vi "Copy Builds To NIVS Dir.vi"(5 "Files Generated by Build":path[](array[path]), 6 "Top Level/Always Included VIs":path[](array[path]), 7 "Destination Path":path, 8 "error in (no error)":errorcluster, 9 "Target Name":string, 10 "Build Specification Name":string, 11 "Project Path":path) -> (0 "error out":errorcluster)   [LabVIEW 2024]
uses:
  <vilib>/Utility/sysdir.llb/System Directory Type.ctl
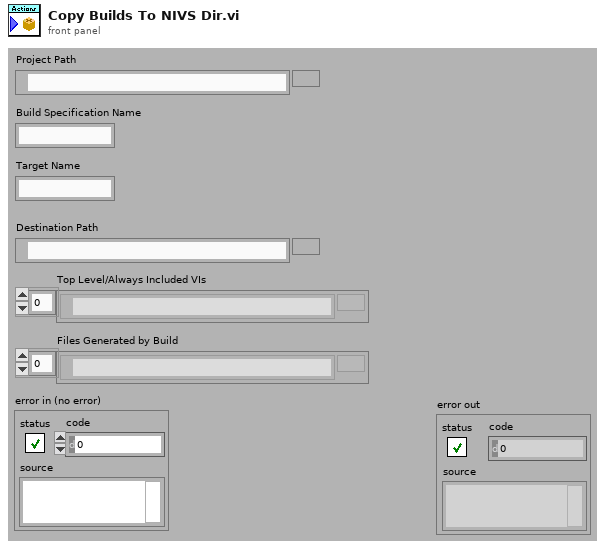
[diagram p1: front panel]
types:
  T1 = typedef "System Directory Type.ctl" = i32
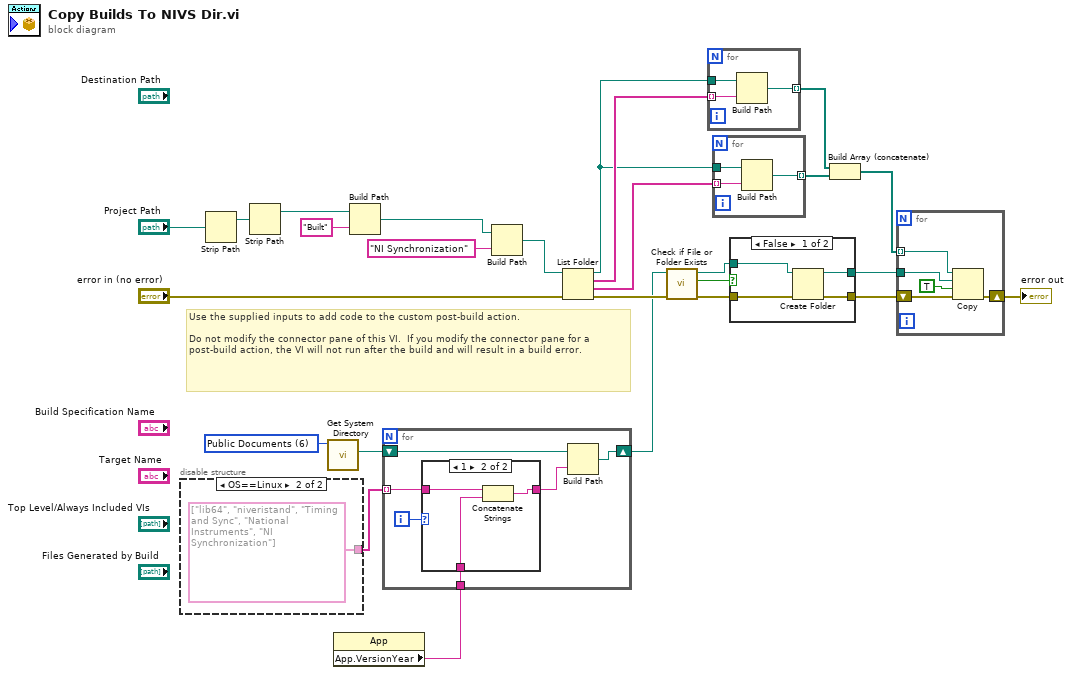
[diagram p0: block diagram]
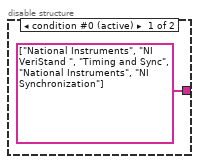
[diagram p2: hidden frame]
diagram:
  w7 = T1 6 items=["User Home"=0, "User Desktop"=1, "User Documents"=2, "User Application Data"=3, "User Preferences"=4, "User Temporary"=5, "Public Documents"=6, "Public Application Data"=7, "Public Preferences"=8, "Public Cache"=13, "System Core Libraries"=9, "System Installed Libraries"=10, "Application Files"=11, "Boot Volume Root"=12] ("system directory type")
  # "Use the supplied inputs to add code to the custom post-build action.\n\nDo not modify the connector pane of this VI.  If you modify the connector pane for a post-build action, the VI will not run after the build and will result in a build error."
  n1 = disable-structure shown="OS==Linux" {
    disable-tunnel: [string[] ["National Instruments", "NI VeriStand ", "Timing and Sync", "National Instruments", "NI Synchronization"] string[] ["lib64", "niveristand", "Timing and Sync", "National Instruments", "NI Synchronization"]] -> w5
    frame condition #0 (active) {
    }
    frame condition #1 {
    }
  }
  n2 = Strip Path(path="Project Path") -> (stripped path=w11:path)  [unwired: 1 out]
  n3 = Strip Path(path=w11) -> (stripped path=w22:path)  [unwired: 1 out]
  n4 = call <vilib>:"Get System Directory.vi"("system directory type"=w7) -> ("system directory"=w6:path)  [unwired: 10 in]
  n5 = property class="App"() -> ("App.VersionYear"=w3:string)  [unwired: 2 in, 2 out]
  n6 = Build Path(base path=w22, name or relative path="Built") -> (appended path=w2:path)
  n7 = for {
    shift-right: [w33] -> w4
    shift-left: w6 -> [w34]
    tunnel: w5 -> [w30] mode=indexing
    tunnel: w3 -> [w29]
    i -> [w32]
    n8 = case shown="1" w32 {
      tunnel: [w35 w37] -> w31
      tunnel: w30 -> [w35 w38]
      tunnel: w29 -> [_ w36]
      frame Default {
      }
      frame 1 {
        n9 = Concatenate Strings(w38, w36) -> (w37:string)
      }
    }
    n10 = Build Path(base path=w34, name or relative path=w31) -> (appended path=w33:path)
  }
  n11 = Build Path(base path=w2, name or relative path="NI Synchronization") -> (appended path=w10:path)
  n12 = List Folder(path=w10, error in="error in (no error)") -> (path out=w13:path, filenames=w26:string[], folder names=w14:string[], error out=w8:errorcluster)  [unwired: 2 in]
  n13 = call <vilib>:"Check if File or Folder Exists.vi"("error in (no error)"=w8, "path"=w4) -> ("error out"=w17:errorcluster, "file or folder exists?"=w19:bool, "dup path"=w18:path)  [unwired: 7 in]
  n14 = for {
    tunnel: w26 -> [w40] mode=indexing
    tunnel: w13 -> [w41]
    tunnel: [w39] -> w25 mode=indexing
    n15 = Build Path(base path=w41, name or relative path=w40) -> (appended path=w39:path)
  }
  n16 = for {
    tunnel: w14 -> [w43] mode=indexing
    tunnel: w13 -> [w44]
    tunnel: [w42] -> w12 mode=indexing
    n17 = Build Path(base path=w44, name or relative path=w43) -> (appended path=w42:path)
  }
  n18 = case shown="False" w19 {
    tunnel: w18 -> [w48 w50]
    tunnel: w17 -> [w47 w49]
    tunnel: [w46 w50] -> w16
    tunnel: [w45 w49] -> w15
    frame False {
      n19 = Create Folder(path (use dialog)=w48, error in=w47) -> (created path=w46:path, error out=w45:errorcluster)  [unwired: 1 in, 1 out]
    }
    frame True {
    }
  }
  n20 = Build Array (concatenate)(w25, w12) -> (w24:path[])
  n21 = for {
    tunnel: w24 -> [w52] mode=indexing
    shift-right: [w53] -> w1
    shift-left: w15 -> [w54]
    tunnel: w16 -> [w51]
    n22 = Copy(8:w54, 9:TRUE ("overwrite (F)"), 10:w51, 11:w52) -> (0:w53:errorcluster)  [unwired: 1 in, 2 out]
  }
  "error out" <- w1
